vi "onHttpPatch (File).vi"(6 "timeout":i32=10000, 7 "output file":path, 8 "error in":errorcluster, 9 "file":path, 10 "url":string, 11 "REST Client in":refnum<class "REST Client.lvclass">) -> (0 "error out":errorcluster, 1 "body":string, 2 "headers":string, 3 "REST Client out":refnum<class "REST Client.lvclass">)   [LabVIEW 2020, in "REST Client.lvlib" / "REST Client.lvclass"]
uses:
  REST Client.lvclass
  REST Client.lvclass/REST Client.ctl
  http-client/http-client.lvclass
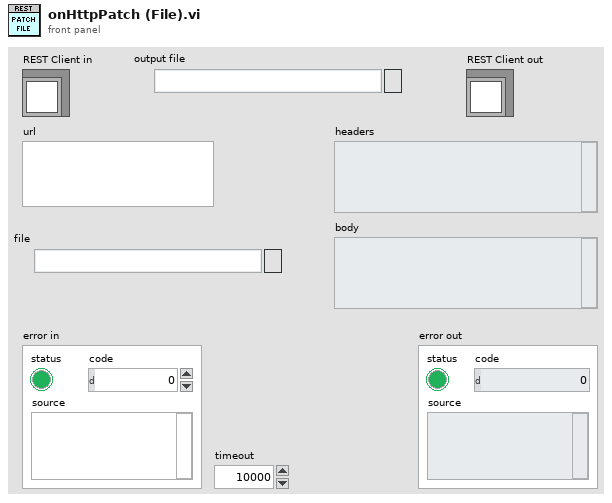
[diagram p1: front panel]
types:
  T1 = typedef "REST Client.lvlib/REST Client.lvclass/HTTP Header.ctl" = cluster{"header":T2, "value":string}
  T2 = typedef "lib_NI_Advanced HTTP Client.lvlib/Session.lvclass/Header--Combo Box.ctl" = string
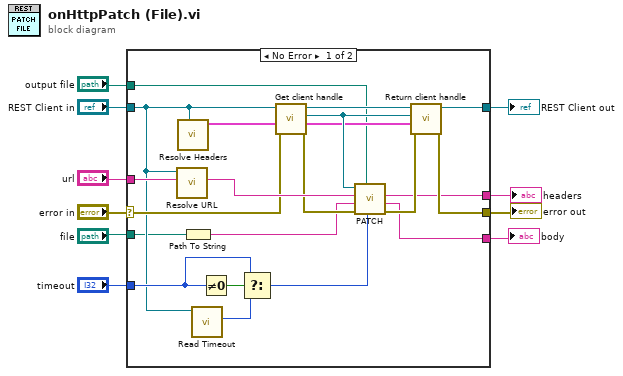
[diagram p0: block diagram]
diagram:
  n1 = case shown="No Error" "error in" {
    selector: "error in" -> [w20 w33]
    tunnel: [w16 w33] -> w2
    tunnel: [w17 w32] -> w4
    tunnel: "REST Client in" -> [w19 w32]
    tunnel: "url" -> [w28 _]
    tunnel: "timeout" -> [w25 _]
    tunnel: [w15 _] -> w3
    tunnel: [w14 _] -> w1
    tunnel: "output file" -> [w13 _]
    tunnel: "file" -> [w12 _]
    frame No Error {
      n2 = call "Resolve URL.vi"("Path"=w28, "REST Client in"=w19) -> ("Resolved URL"=w27:string)  [unwired: 9 in]
      n3 = call "Resolve Headers.vi"("REST Client in"=w19) -> ("headers out"=w18:T1[])  [unwired: 10 in]
      n4 = Path To String(path=w12) -> (string=w11:string)
      n5 = call-dynamic "Read Timeout.vi"("REST Client in"=w19) -> ("Timeout"=w22:i32)  [unwired: 8 in, 2 out]
      n6 = Not Equal To 0?(x=w25) -> (x != 0?=w26:bool)
      n7 = Select(t=w25, s=w26, f=w22) -> (s? t:f=w24:i32)
      n8 = call "Get client handle.vi"("error in (no error)"=w20, "headers"=w18, "REST Client in"=w19) -> ("error out"=w23:errorcluster, "headers out"=w29:T1[], "http-client"=w30:refnum<class "http-client.lvclass">, "REST Client out"=w31:refnum<class "REST Client.lvclass">)  [unwired: 5 in]
      n9 = call "PATCH.vi"("timeout"=w24, "output file"=w13, "error in"=w23, "buffer"=w11, "url"=w27, "http-client in"=w30) -> ("error out"=w21:errorcluster, "body"=w14:string, "headers"=w15:string)  [unwired: 1 in, 2 out]
      n10 = call "Return client handle.vi"("error in (no error)"=w21, "headers"=w29, "http-client"=w30, "REST Client in"=w31) -> ("error out"=w16:errorcluster, "REST Client out"=w17:refnum<class "REST Client.lvclass">)  [unwired: 6 in]
    }
    frame Error {
    }
  }
  "error out" <- w2
  "REST Client out" <- w4
  "headers" <- w3
  "body" <- w1
